vi "ZM-ROOT-notePackageType.vi"(8 "error in (no error)":errorcluster, 10 "package":refnum<class "ZM-PC-package.lvclass">, 11 "ZM-ROOT-root in":refnum<class "ZM-ROOT-root.lvclass">) -> (0 "error out":errorcluster, 3 "ZM-ROOT-root out":refnum<class "ZM-ROOT-root.lvclass">)   [LabVIEW 2020, in "ZM-ROOT-root.lvlib" / "ZM-ROOT-root.lvclass"]
doc: "Member of the root (static, private), called by ZM-CI-handlePackage for a package to Communication and for a non-error package to Root: Read type -> Write lastPackageType; Read packageCount -> +1 -> Write packageCount. One error chain."
uses:
  ZM-ROOT-root.lvclass
  common/ZM-PC-packages/ZM-PC-package/ZM-PC-package.lvclass
  ZM-ROOT-root.lvclass/ZM-ROOT-root.ctl
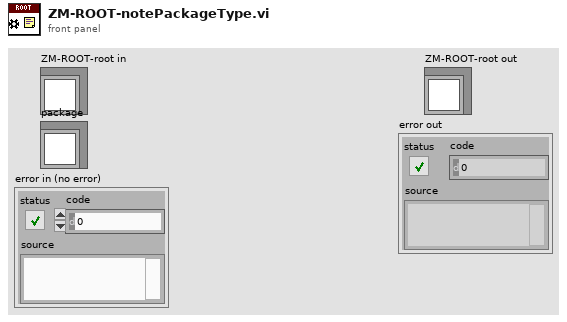
[diagram p1: front panel]
types:
  T1 = typedef "ZM-PC-packages.lvlib/ZM-PC-package.lvclass/ZM-PC-PACKAGE_TYPE.ctl" = enum16{"Undefined", "TestPackage", "ErrorPackage"}
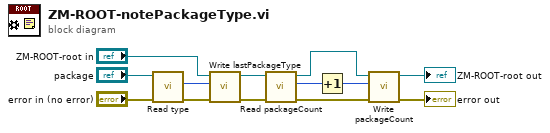
[diagram p0: block diagram]
diagram:
  n1 = call "Read type.vi"("error in (no error)"="error in (no error)", "ZM-PC-package in"="package") -> ("error out"=w11:errorcluster, "ZM-PC-PACKAGE_TYPE"=w9:T1)  [unwired: 7 in, 1 out]
  n2 = call "Write lastPackageType.vi"("error in (no error)"=w11, "ZM-PC-PACKAGE_TYPE"=w9, "ZM-ROOT-root in"="ZM-ROOT-root in") -> ("error out"=w8:errorcluster, "ZM-ROOT-root out"=w7:refnum<class "ZM-ROOT-root.lvclass">)  [unwired: 7 in]
  n3 = call "Read packageCount.vi"("error in (no error)"=w8, "ZM-ROOT-root in"=w7) -> ("error out"=w5:errorcluster, "packageCount"=w6:u32, "ZM-ROOT-root out"=w4:refnum<class "ZM-ROOT-root.lvclass">)  [unwired: 7 in]
  n4 = Increment(x=w6) -> (x+1=w3:u32)
  n5 = call "Write packageCount.vi"("error in (no error)"=w5, "packageCount"=w3, "ZM-ROOT-root in"=w4) -> ("error out"=→"error out":errorcluster, "ZM-ROOT-root out"=→"ZM-ROOT-root out":refnum<class "ZM-ROOT-root.lvclass">)  [unwired: 7 in]
